vi "CSE - Link Source Script Line to Statements.vi"(8 "error in":errorcluster, 10 "Line number (1)":i32=1, 11 "CSE RefNum":T1) -> (0 "error out":errorcluster, 1 "Stm Indexes":i32[](array[numeric]), 2 "dup Line number":i32=1, 3 "dup CSE RefNum":T1)   [LabVIEW 2021]
doc: "This VI returns the indexes of statements in a parsed script that start on the specified line of the source script. If no statement starts on the specified line, the VI returns an empty array of statement indexes. The line numbers start at 1. Refer to the VI help for more details.\n\n::: CalcExpress Toolkit :::\nCopyright (c) 2000-2026 Konstantin Shifershteyn. All rights reserved."
uses:
  CSE Instance RefNum.ctl
  cersrc/celveng32.dll
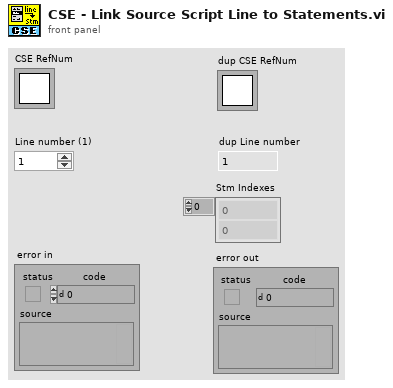
[diagram p1: front panel]
types:
  T1 = typedef "CSE Instance RefNum.ctl" = refnum<k1>
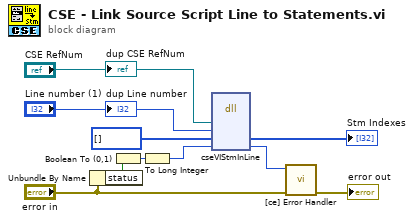
[diagram p0: block diagram]
diagram:
  n1 = Unbundle By Name("error in") -> ("status"=w9:bool)
  n2 = Boolean To (0,1)(Boolean=w9) -> (0, 1=w10:i16)
  n3 = To Long Integer(number=w10) -> (32bit integer=w6:i32)
  n4 = dll-call lib="C:/LV Projects/CalcExpress 40 LV2021/vi.lib/addons/CalcExpress/cersrc/celveng*.dll" fn="cseVIStmInLine"("iCESP"="CSE RefNum", "LineNumber"="Line number (1)", "StmIdxArray"=i32[] [], "errStat"=w6) -> ("StmIdxArray"=→"Stm Indexes":i32[], "errStat"=w5:i32)  [unwired: 6 in, 2 out]
  n5 = call "[ce] Error Handler.vi"("error in"="error in", "error code"=w5) -> ("error out"=→"error out":errorcluster)  [unwired: 8 in, 1 out]
  "dup CSE RefNum" <- "CSE RefNum"
  "dup Line number" <- "Line number (1)"
